vi "Initialize App.vi"() -> (0 "error out":errorcluster, 1 "notifier cluster":T1, 2 "Stop Event":refnum<user-event>, 3 "queue cluster":T2)   [LabVIEW 2021]
uses:
  Type defs/Queues.ctl
  Type defs/Message cluster.ctl
  Type defs/Notifiers.ctl
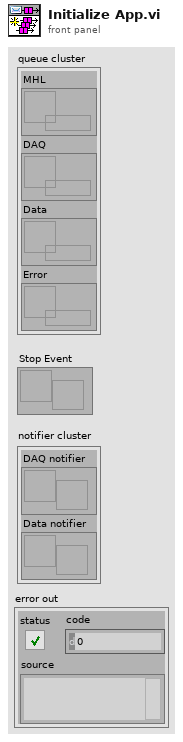
[diagram p1: front panel]
types:
  T1 = typedef "Notifiers.ctl" = cluster{"DAQ notifier":refnum<notifier>, "Data notifier":refnum<notifier>}
  T2 = typedef "Queues.ctl" = cluster{"MHL":refnum<queue>, "DAQ":refnum<queue>, "Data":refnum<queue>, "Error":refnum<queue>}
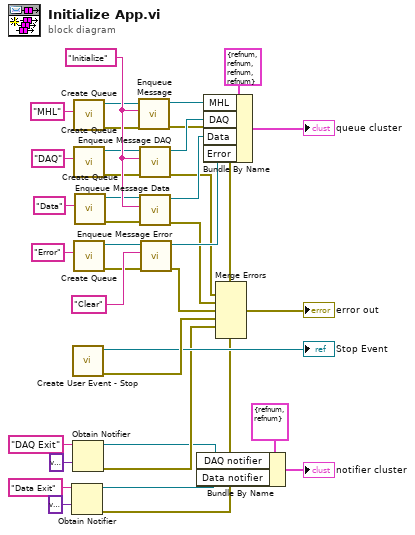
[diagram p0: block diagram]
diagram:
  w33 = "Initialize"
  n1 = Obtain Notifier(name (unnamed)="Data Exit", notification data type=variant ("element data type")) -> (notifier out=w2:refnum<notifier>, error out=w7:errorcluster)  [unwired: 2 in, 1 out]
  n2 = call "Create User Event - Stop.vi"() -> ("error out"=w14:errorcluster, "Stop Event"=→"Stop Event":refnum<user-event>)  [unwired: 10 in]
  n3 = Obtain Notifier(name (unnamed)="DAQ Exit", notification data type=variant ("element data type")) -> (notifier out=w3:refnum<notifier>, error out=w8:errorcluster)  [unwired: 2 in, 1 out]
  n4 = call "Create Queue.vi"("name (unnamed)"="MHL") -> ("error out"=w24:errorcluster, "queue out"=w31:refnum<queue>)  [unwired: 9 in]
  n5 = call "Create Queue.vi"("name (unnamed)"="DAQ") -> ("error out"=w25:errorcluster, "queue out"=w30:refnum<queue>)  [unwired: 9 in]
  n6 = call "Create Queue.vi"("name (unnamed)"="Error") -> ("error out"=w27:errorcluster, "queue out"=w28:refnum<queue>)  [unwired: 9 in]
  n7 = call "Create Queue.vi"("name (unnamed)"="Data") -> ("error out"=w26:errorcluster, "queue out"=w29:refnum<queue>)  [unwired: 9 in]
  n8 = call "Enqueue Message.vi"("error in (no error)"=w24, "Message"=w33, "queue in"=w31) -> ("error out"=w18:errorcluster, "queue out"=w23:refnum<queue>)  [unwired: 7 in]
  n9 = call "Enqueue Message DAQ.vi"("error in (no error)"=w25, "Message"=w33, "queue in"=w30) -> ("error out"=w17:errorcluster, "queue out"=w21:refnum<queue>)  [unwired: 7 in]
  n10 = call "Enqueue Message Data.vi"("error in (no error)"=w26, "Message"=w33, "queue in"=w29) -> ("error out"=w16:errorcluster, "queue out"=w20:refnum<queue>)  [unwired: 7 in]
  n11 = call "Enqueue Message Error.vi"("error in (no error)"=w27, "Message"="Clear", "queue in"=w28) -> ("error out"=w15:errorcluster, "queue out"=w19:refnum<queue>)  [unwired: 7 in]
  n12 = Bundle By Name(cluster=T1 {"DAQ notifier"=refnum, "Data notifier"=refnum} ("notifier cluster"), "DAQ notifier"=w3, "Data notifier"=w2) -> (→"notifier cluster":T1)
  n13 = Bundle By Name(cluster=T2 {"MHL"=refnum, "DAQ"=refnum, "Data"=refnum, "Error"=refnum} ("Queues"), "MHL"=w23, "DAQ"=w21, "Data"=w20, "Error"=w19) -> (→"queue cluster":T2)
  n14 = Merge Errors(w18, w17, w16, w15, w14, w8, w7) -> (→"error out":errorcluster)
